vi "FRC Hack Build Path.vi"(8 "error in (no error)":errorcluster, 9 "new path":path, 10 "build spec name":string, 11 "TargetItem Refnum":refnum<vi>) -> (0 "error out":errorcluster)   [LabVIEW 2025]
uses:
  <resource>/Framework/Providers/API/mxLvNIIM.ctl
  <vilib>/AppBuilder/AB_Relative_Path_Type.ctl
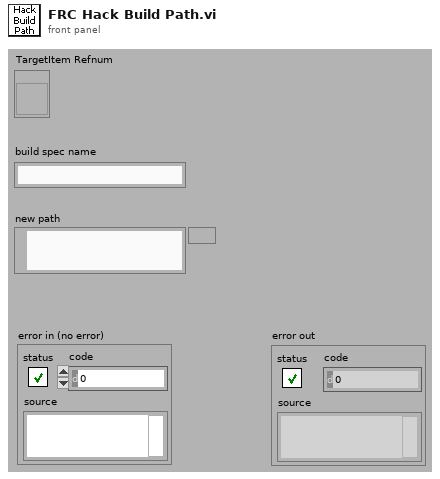
[diagram p1: front panel]
types:
  T1 = typedef "AB_Relative_Path_Type.ctl" = enum16{"<none>", "relativeToCommon", "relativeToAppDir", "relativeToProject", "relativeToLabVIEWData"}
  T2 = typedef "mxLvNIIM.ctl" = cluster{"Item URL":string, "Item ID":string, "Item Index":i32, "Specific Type":string}
  T3 = typedef "ItemRef.ctl" = u64
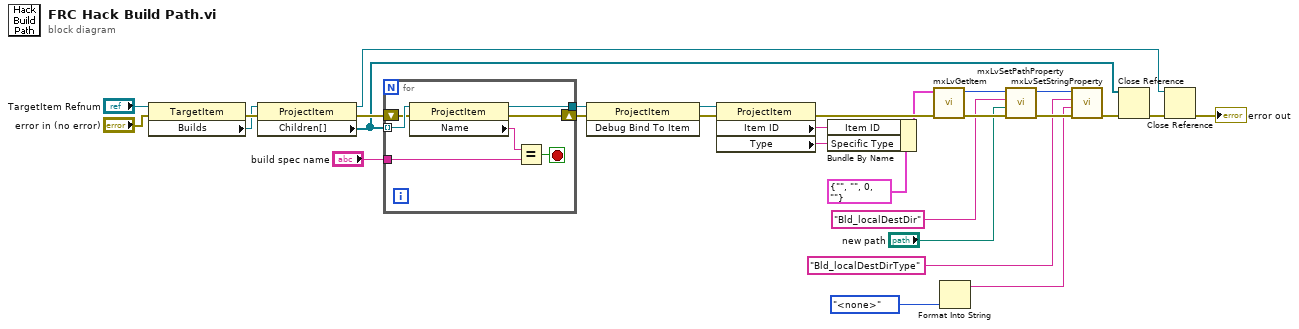
[diagram p0: block diagram]
diagram:
  n1 = property class="TargetItem"(reference="TargetItem Refnum", error in="error in (no error)") -> (error out=w6:errorcluster, "Builds"=w5:refnum<vi>)  [unwired: 1 out]
  n2 = property class="ProjectItem"(reference=w5, error in=w6) -> (reference out=w20:refnum<vi>, error out=w27:errorcluster, "Children[]"=w21:refnum<vi>[])
  n3 = for {
    tunnel: w21 -> [w36] mode=indexing
    tunnel: "build spec name" -> [w34]
    shift-right: [w31] -> w2
    shift-left: w27 -> [w32]
    tunnel: [w30] -> w4
    stop <- w33 stop-if-true
    n4 = property class="ProjectItem"(reference=w36, error in=w32) -> (reference out=w30:refnum<vi>, error out=w31:errorcluster, "Name"=w35:string)
    n5 = Equal?(x=w35, y=w34) -> (x = y?=w33:bool)
  }
  n6 = invoke class="ProjectItem" method="Debug Bind To Item"(reference=w4, error in=w2) -> (reference out=w3:refnum<vi>, error out=w1:errorcluster)  [unwired: 1 in, 1 out]
  n7 = property class="ProjectItem"(reference=w3, error in=w1) -> (error out=w23:errorcluster, "Item ID"=w24:string, "Type"=w7:string)  [unwired: 1 out]
  n8 = Bundle By Name(cluster=T2 {"Item URL"="", "Item ID"="", "Item Index"=0, "Specific Type"=""} ("NIIM"), "Item ID"=w24, "Specific Type"=w7) -> (w22:T2)
  n9 = call <resource>:"mxLvGetItem.vi"("error in"=w23, "NIIM"=w22) -> ("error out"=w16:errorcluster, "Item"=w17:T3)  [unwired: 8 out]
  n10 = Format Into String(AB_Relative_Path_Type."<none>" ("relativeType")) -> (resulting string=w8:string)  [unwired: 3 in, 1 out]
  n11 = call <resource>:"mxLvSetPathProperty.vi"("error in"=w16, "Path"="new path", "Tag"="Bld_localDestDir", "Item"=w17) -> ("error out"=w14:errorcluster, "Item"=w12:T3)  [unwired: 1 in, 5 out]
  n12 = call <resource>:"mxLvSetStringProperty.vi"("error in"=w14, "Value (\"\")"=w8, "Tag"="Bld_localDestDirType", "Item"=w12) -> ("error out"=w13:errorcluster)  [unwired: 1 in, 6 out]
  n13 = Close Reference(reference=w21, error in (no error)=w13) -> (error out=w19:errorcluster)
  n14 = Close Reference(reference=w20, error in (no error)=w19) -> (error out=→"error out":errorcluster)
